vi "RemoteVI App Alarms.vi"() -> ()   [LabVIEW 2020]
doc: "Screen Alarms of RemoteVI Application Example.vi: active alarms of the station (simulated: a new one arrives every 6 s while fewer than 10 are active). Acknowledge removes the selected alarm, Acknowledge All every alarm. Runs until the notifier RemoteVI Application Example fires (the main VI quits)."
panel:
  out "Alarm":bool
  out "Active Alarms":i32
  in  "Acknowledge All":bool
  in  "Acknowledge":bool
  in  "Alarms":i32(listbox)=-1
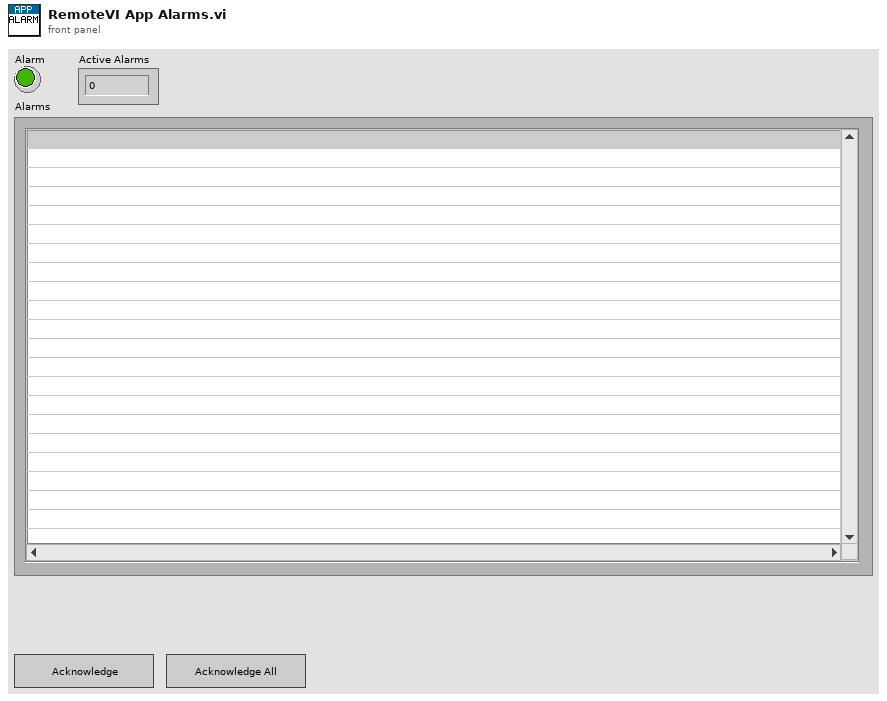
[diagram p1: front panel]
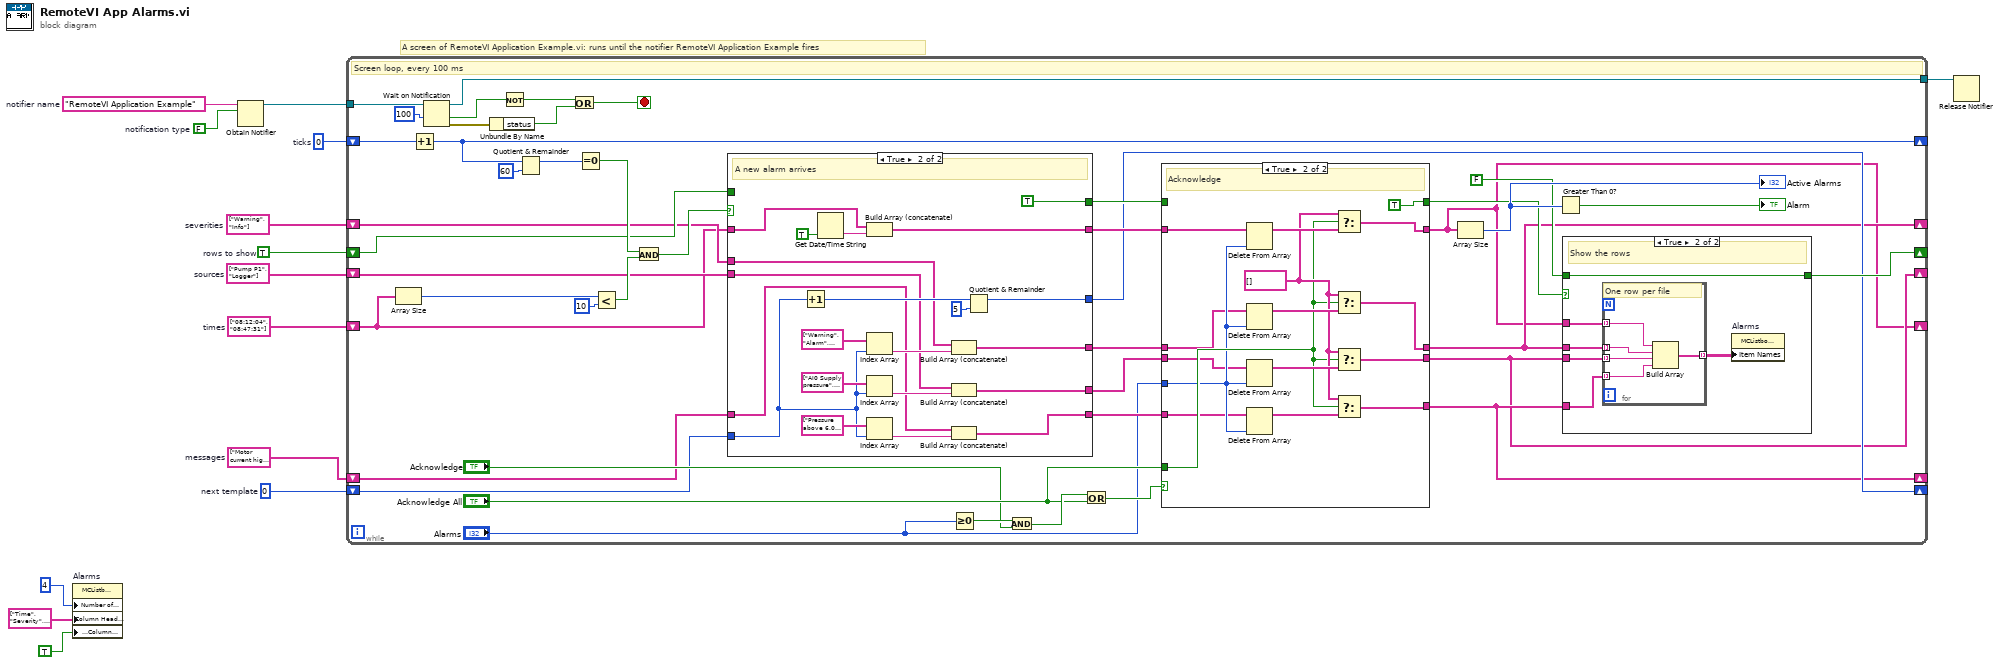
[diagram p0: block diagram]
diagram:
  w9 = FALSE  # notification type
  w8 = "RemoteVI Application Example"  # notifier name
  w7 = TRUE  # rows to show
  w6 = 0  # next template
  w5 = 0  # ticks
  w4 = string[] ["Motor current high", "Log file split"]  # messages
  w3 = string[] ["Pump P1", "Logger"]  # sources
  w2 = string[] ["Warning", "Info"]  # severities
  w1 = string[] ["08:12:04", "08:47:31"]  # times
  # "A screen of RemoteVI Application Example.vi: runs until the notifier RemoteVI Application Example fires"
  n1 = property on="Alarms" class="MCListbox (strict)"("Number of Columns"=4, "Column Header Strings[]"=string[] ["Time", "Severity", "Source", "Message"], "Visible Items:Column Headers Visible"=TRUE) -> ()  [unwired: 2 in, 2 out]
  n2 = Obtain Notifier(name (unnamed)=w8, notification data type=w9) -> (notifier out=w10:refnum<notifier>)  [unwired: 2 in, 2 out]
  n3 = while {
    shift-right: [w17] -> _
    shift-left: w1 -> [w16]
    shift-right: [w19] -> _
    shift-left: w2 -> [w18]
    shift-right: [w21] -> _
    shift-left: w3 -> [w20]
    shift-right: [w23] -> _
    shift-left: w4 -> [w22]
    shift-right: [w25] -> _
    shift-left: w5 -> [w24]
    shift-right: [w27] -> _
    shift-left: w6 -> [w26]
    shift-right: [w29] -> _
    shift-left: w7 -> [w28]
    tunnel: w10 -> [w15]
    tunnel: [w53] -> w14
    stop <- w58 stop-if-true
    # "Screen loop, every 100 ms"
    n4 = Array Size(array=w16) -> (size(s)=w36:i32)
    n5 = Increment(x=w24) -> (x+1=w25:i32)
    n6 = Wait on Notification(notifier=w15, timeout in ms (-1)=100) -> (notifier out=w53:refnum<notifier>, timed out?=w54:bool, error out=w55:errorcluster)  [unwired: 2 in, 1 out]
    n7 = Unbundle By Name(w55) -> ("status"=w57:bool)
    n8 = Not(x=w54) -> (.not. x?=w56:bool)
    n9 = Quotient & Remainder(x=w25, y=60) -> (x-y*floor(x/y)=w34:i32)  [unwired: 1 out]
    n10 = Or(x=w56, y=w57) -> (x .or. y?=w58:bool)
    n11 = Equal To 0?(x=w34) -> (x = 0?=w35:bool)
    n12 = Less?(x=w36, y=10) -> (x < y?=w38:bool)
    n13 = And(x=w35, y=w38) -> (x .and. y?=w39:bool)
    n14 = case shown="True" w39 {
      tunnel: w16 -> [w92 w98]
      tunnel: w18 -> [w93 w99]
      tunnel: w20 -> [w94 w100]
      tunnel: w22 -> [w95 w101]
      tunnel: w26 -> [w96 w102]
      tunnel: w28 -> [w97 _]
      tunnel: [w92 w111] -> w40
      tunnel: [w93 w112] -> w41
      tunnel: [w94 w113] -> w42
      tunnel: [w95 w114] -> w43
      tunnel: [w96 w117] -> w27
      tunnel: [w97 TRUE] -> w44
      frame False {
        # "No new alarm"
      }
      frame True {
        # "A new alarm arrives"
        n15 = Increment(x=w102) -> (x+1=w115:i32)
        n16 = Get Date/Time String(want seconds? (F)=TRUE) -> (time string=w104:string)  [unwired: 3 out]
        n17 = Build Array (concatenate)(w98, w104) -> (w111:string[])
        n18 = Index Array(array=string[] ["Warning", "Alarm", "Warning", "Alarm", "Info"], index=w102) -> (element=w106:string)
        n19 = Index Array(array=string[] ["AI0 Supply pressure", "AI2 Coolant temperature", "Pump P1", "AI3 Flow", "Logger"], index=w102) -> (element=w108:string)
        n20 = Index Array(array=string[] ["Pressure above 6.0 bar", "Temperature above 45 degC", "Motor current high", "Flow below 2 l/min", "Disk space below 10 %"], index=w102) -> (element=w110:string)
        n21 = Build Array (concatenate)(w99, w106) -> (w112:string[])
        n22 = Build Array (concatenate)(w100, w108) -> (w113:string[])
        n23 = Build Array (concatenate)(w101, w110) -> (w114:string[])
        n24 = Quotient & Remainder(x=w115, y=5) -> (x-y*floor(x/y)=w117:i32)  [unwired: 1 out]
      }
    }
    n25 = Greater Or Equal To 0?(x="Alarms") -> (x >= 0?=w45:bool)
    n26 = And(x=w45, y="Acknowledge") -> (x .and. y?=w46:bool)
    n27 = Or(x=w46, y="Acknowledge All") -> (x .or. y?=w47:bool)
    n28 = case shown="True" w47 {
      tunnel: "Alarms" -> [_ w80]
      tunnel: "Acknowledge All" -> [_ w81]
      tunnel: w40 -> [w71 w76]
      tunnel: w41 -> [w72 w77]
      tunnel: w42 -> [w73 w78]
      tunnel: w43 -> [w74 w79]
      tunnel: w44 -> [w75 _]
      tunnel: [w71 w84] -> w17
      tunnel: [w72 w86] -> w19
      tunnel: [w73 w88] -> w21
      tunnel: [w74 w90] -> w23
      tunnel: [w75 TRUE] -> w48
      frame False {
        # "Nothing to acknowledge"
      }
      frame True {
        w82 = string[] []
        # "Acknowledge"
        n29 = Delete From Array(array=w76, index=w80) -> (array with subset deleted=w83:string[])  [unwired: 1 in, 1 out]
        n30 = Delete From Array(array=w77, index=w80) -> (array with subset deleted=w85:string[])  [unwired: 1 in, 1 out]
        n31 = Delete From Array(array=w78, index=w80) -> (array with subset deleted=w87:string[])  [unwired: 1 in, 1 out]
        n32 = Delete From Array(array=w79, index=w80) -> (array with subset deleted=w89:string[])  [unwired: 1 in, 1 out]
        n33 = Select(t=w82, s=w81, f=w83) -> (s? t:f=w84:string[])
        n34 = Select(t=w82, s=w81, f=w85) -> (s? t:f=w86:string[])
        n35 = Select(t=w82, s=w81, f=w87) -> (s? t:f=w88:string[])
        n36 = Select(t=w82, s=w81, f=w89) -> (s? t:f=w90:string[])
      }
    }
    n37 = Array Size(array=w17) -> (size(s)=w50:i32)
    "Active Alarms" <- w50
    n38 = Greater Than 0?(x=w50) -> (x > 0?=→"Alarm":bool)
    n39 = case shown="True" w48 {
      tunnel: FALSE -> [w59 w64]
      tunnel: [w59 w64] -> w29
      tunnel: w17 -> [_ w60]
      tunnel: w19 -> [_ w61]
      tunnel: w21 -> [_ w62]
      tunnel: w23 -> [_ w63]
      frame False {
        # "Rows unchanged"
      }
      frame True {
        # "Show the rows"
        n40 = for {
          tunnel: w60 -> [w66] mode=indexing
          tunnel: w61 -> [w67] mode=indexing
          tunnel: w62 -> [w68] mode=indexing
          tunnel: w63 -> [w69] mode=indexing
          tunnel: [w70] -> w65 mode=indexing
          # "One row per file"
          n41 = Build Array(w66, w67, w68, w69) -> (w70:string[])
        }
        n42 = property on="Alarms" class="MCListbox (strict)"("Item Names"=w65) -> ()  [unwired: 2 in, 2 out]
      }
    }
  }
  n43 = Release Notifier(notifier=w14) -> ()  [unwired: 2 in, 3 out]
